vi "BNAL TDMS save table_MS.vi"(8 "error in":errorcluster caption="エラー入力（エラーなし）", 9 "Tag cluster_B":T1, 10 "Table cluster_B":T2, 11 "TDMSファイル入力":refnum<k34>) -> (0 "error out":errorcluster caption="エラー出力", 3 "A TDMSファイル出力":refnum<k34>)   [LabVIEW 2018]
panel:
  out "LAP Table":string[][](table) caption="BS Table"
  out "LAP Table Tag":string[](array[string])
  out "BS Table Tag":string[](array[string])
  out "BS Table":string[][](table)
  out "LTP Table Tag":string[](array[string])
  out "LTP Table":string[][](table)
  out "LCP Table Tag":string[](array[string])
  out "LSP Table Tag":string[](array[string])
  out "LCP Table":string[][](table)
  out "LSP Table":string[][](table)
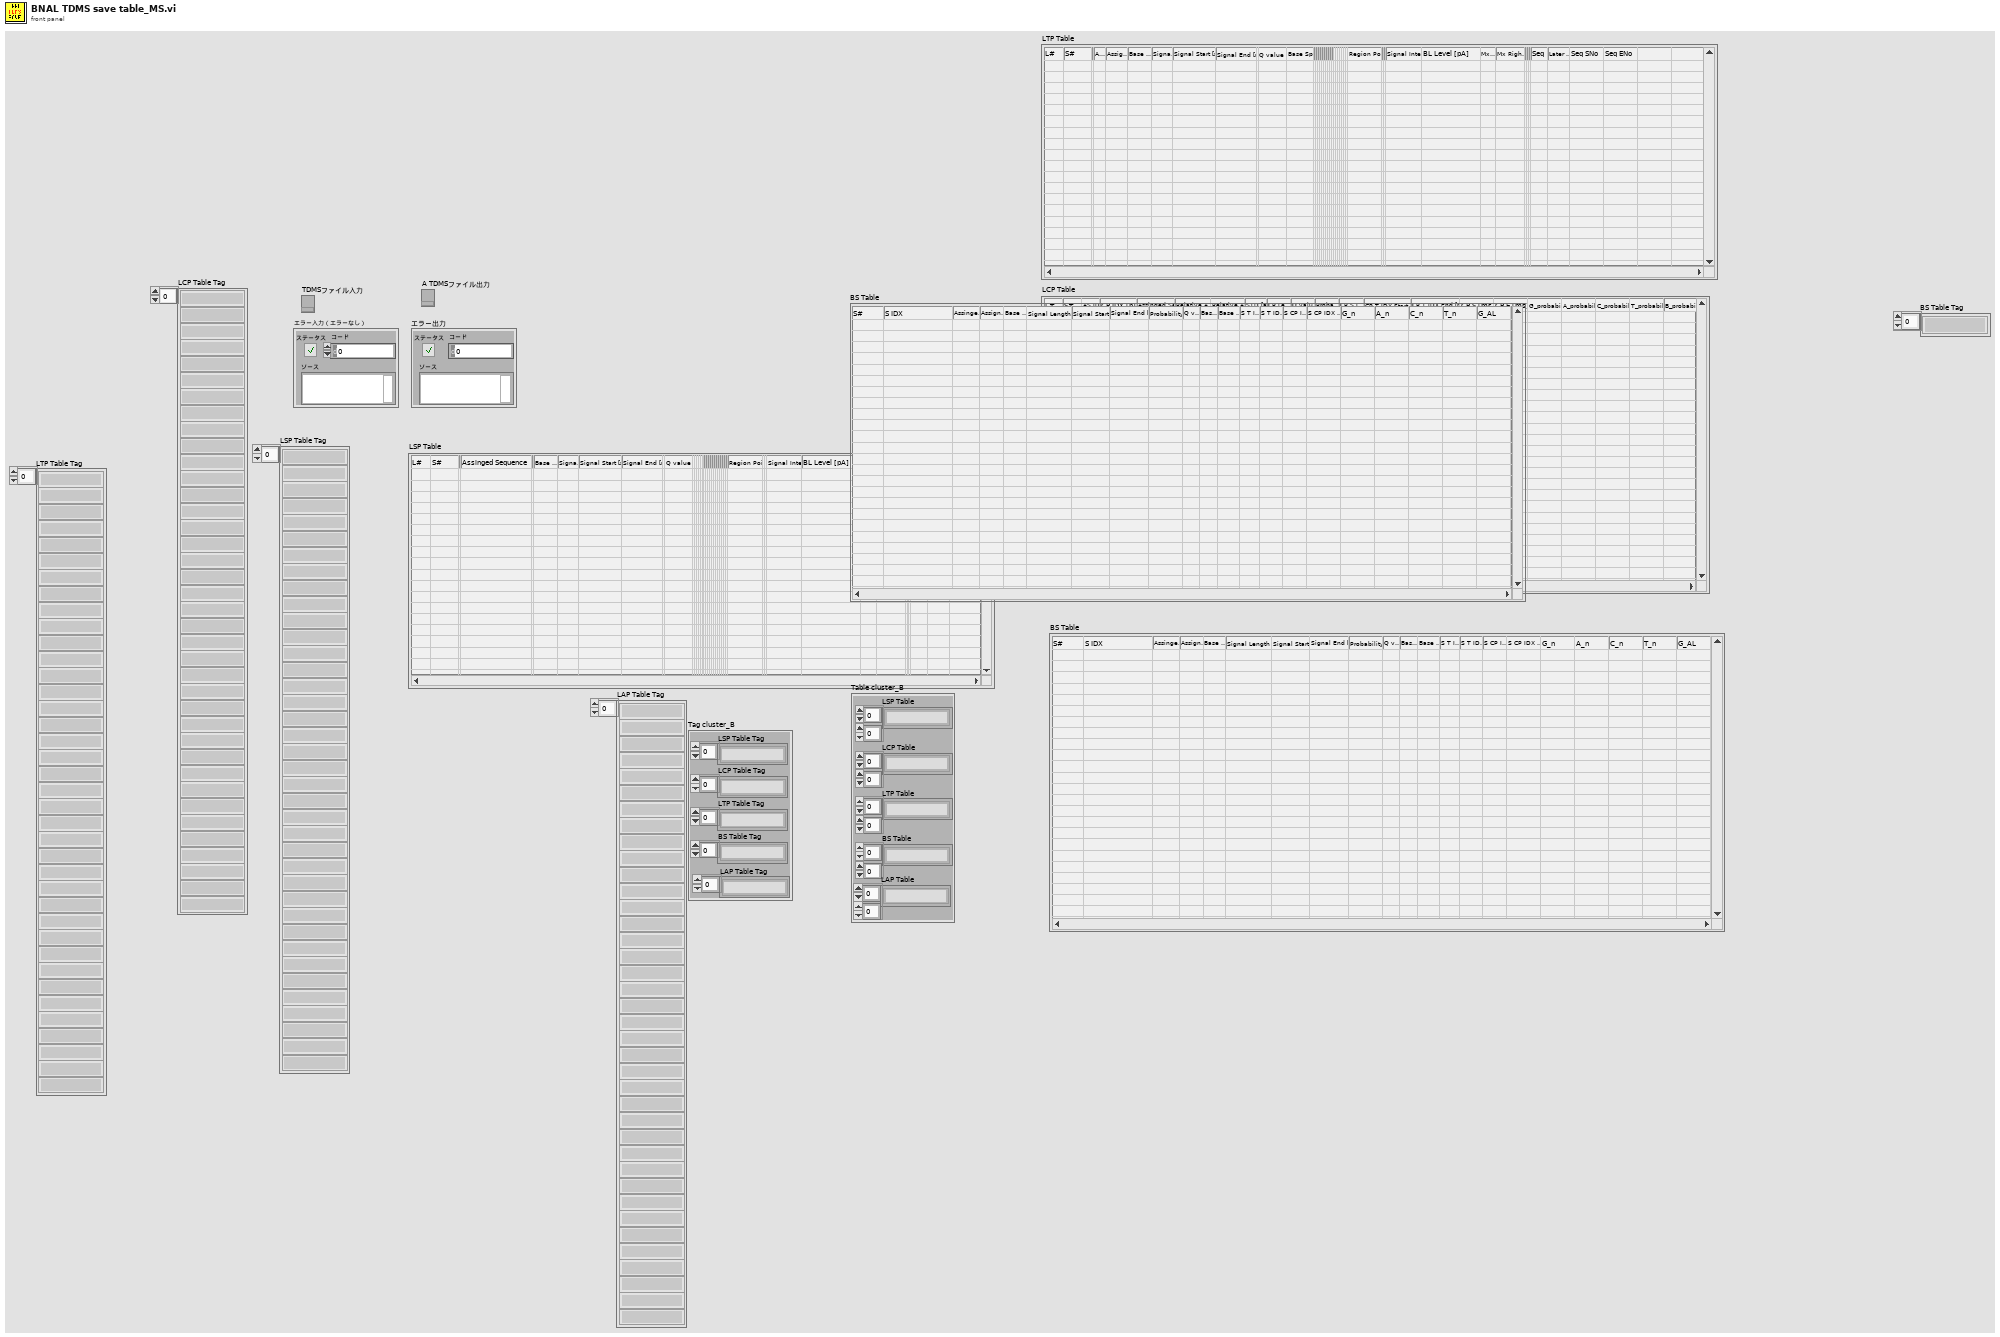
[diagram p1: front panel]
types:
  T1 = cluster{"LSP Table Tag":string[], "LCP Table Tag":string[], "LTP Table Tag":string[], "BS Table Tag":string[], "LAP Table Tag":string[]}
  T2 = cluster{"LSP Table":string[][], "LCP Table":string[][], "LTP Table":string[][], "BS Table":string[][], "LAP Table":string[][]}
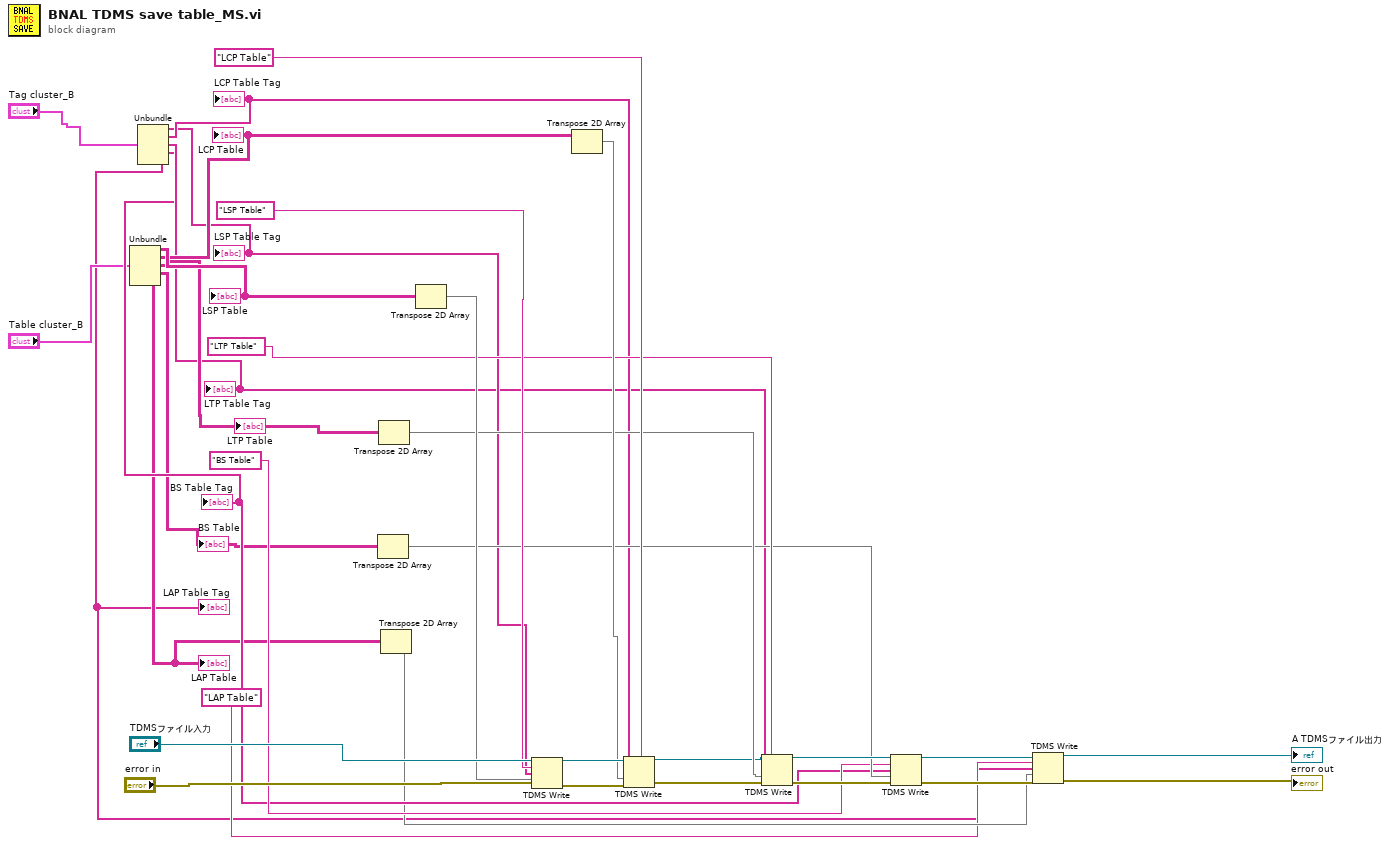
[diagram p0: block diagram]
diagram:
  n1 = Unbundle("Table cluster_B") -> ("LSP Table"=w18:string[][], "LCP Table"=w17:string[][], "LTP Table"=w14:string[][], "BS Table"=w11:string[][], "LAP Table"=w4:string[][])
  "LSP Table" <- w18
  "LCP Table" <- w17
  "LTP Table" <- w14
  "BS Table" <- w11
  "LAP Table" <- w4
  n2 = Unbundle("Tag cluster_B") -> ("LSP Table Tag"=w15:string[], "LCP Table Tag"=w16:string[], "LTP Table Tag"=w13:string[], "BS Table Tag"=w12:string[], "LAP Table Tag"=w1:string[])
  "LSP Table Tag" <- w15
  "LCP Table Tag" <- w16
  "LTP Table Tag" <- w13
  "BS Table Tag" <- w12
  "LAP Table Tag" <- w1
  n3 = Transpose 2D Array(2D array=w11) -> (transposed array=w20:string[][])
  n4 = Transpose 2D Array(2D array=w14) -> (transposed array=w25:string[][])
  n5 = Transpose 2D Array(2D array=w4) -> (transposed array=w3:string[][])
  n6 = Transpose 2D Array(2D array=w18) -> (transposed array=w28:string[][])
  n7 = TDMS Write(0:"TDMSファイル入力", 5:"LSP Table" ("チャンネル名入力（名称未設定）"), 7:w15, 9:w28, 11:"error in") -> (4:w33:refnum<k34>, 15:w34:errorcluster)  [unwired: 1 in, 2 out]
  n8 = Transpose 2D Array(2D array=w17) -> (transposed array=w27:string[][])
  n9 = TDMS Write(0:w33, 5:"LCP Table" ("チャンネル名入力（名称未設定）"), 7:w16, 9:w27, 11:w34) -> (4:w24:refnum<k34>, 15:w26:errorcluster)  [unwired: 1 in, 2 out]
  n10 = TDMS Write(0:w24, 5:"LTP Table" ("チャンネル名入力（名称未設定）"), 7:w13, 9:w25, 11:w26) -> (4:w22:refnum<k34>, 15:w21:errorcluster)  [unwired: 1 in, 2 out]
  n11 = TDMS Write(0:w22, 5:"BS Table" ("チャンネル名入力（名称未設定）"), 7:w12, 9:w20, 11:w21) -> (4:w8:refnum<k34>, 15:w6:errorcluster)  [unwired: 1 in, 2 out]
  n12 = TDMS Write(0:w8, 5:"LAP Table" ("チャンネル名入力（名称未設定）"), 7:w1, 9:w3, 11:w6) -> (4:→"A TDMSファイル出力":refnum<k34>, 15:→"error out":errorcluster)  [unwired: 1 in, 2 out]
